vi "GpuMat IsContinuous.vi"(8 "error in (no error)":errorcluster, 11 "GpuMat in":refnum<class "GpuMat.lvclass">) -> (0 "error out":errorcluster, 2 "IsContinuous":bool, 3 "GpuMat out":refnum<class "GpuMat.lvclass">)   [LabVIEW 2020, in "OpenLvVision_OpenCv.lvlib" / "Cuda.lvlib" / "GpuMat.lvclass"]
doc: "Returns true if the GpuMat is stored contiguously (no padding/gaps between rows)."
uses:
  GpuMat.lvclass
  C:/Users/lukas/Documents/OpenLvVision_OpenCv/SourceCode/LabView/OpenLvVision_OpenCv/_LvHelpers/EdvrObject/EdvrObject.lvclass
  _LvHelpers/EdvrObject/EdvrObject.lvclass/EdvrObject.ctl
  OpenLvVision_OpenCv.lvlib
  <vilib>/Utility/error.llb/Error Cluster From Error Code.vi
  <vilib>/ErrorRing/Error Ring.xnode
  _LvHelpers/EdvrObject/EdvrObject.lvclass
  Dlls/OlvOpenCvWrapper.dll
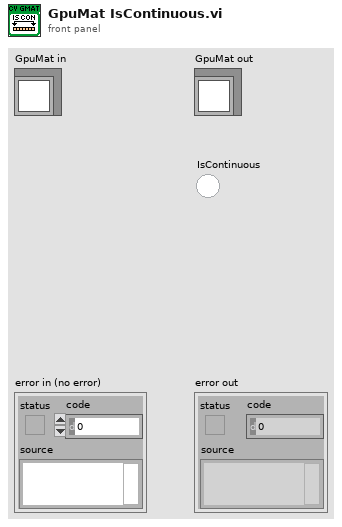
[diagram p1: front panel]
types:
  T1 = typedef "OpenLvVision_OpenCv.lvlib/EdvrObject.lvclass/Edvr.ctl" = refnum<data-value>
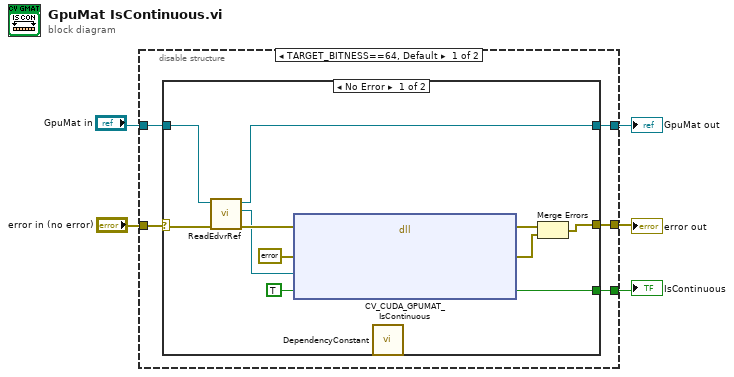
[diagram p0: block diagram]
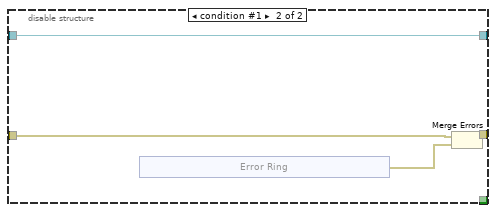
[diagram p3: hidden frame]
diagram:
  n1 = disable-structure shown="TARGET_BITNESS==64, Default" {
    disable-tunnel: "error in (no error)" -> [w10 w26]
    disable-tunnel: [w9 w27] -> w5
    disable-tunnel: "GpuMat in" -> [w8 w24]
    disable-tunnel: [w7 w24] -> w2
    disable-tunnel: [w6 _] -> w1
    frame condition #0 (active) {
      n2 = case shown="No Error" w10 {
        selector: w10 -> [w13 w23]
        tunnel: [w18 w23] -> w9
        tunnel: w8 -> [w16 w22]
        tunnel: [w14 w22] -> w7
        tunnel: [w12 _] -> w6
        frame No Error {
          n3 = call "ReadEdvrRef.vi"("error in (no error)"=w13, "EdvrObject in"=w16) -> ("error out"=w17:errorcluster, "Edvr"=w15:T1, "EdvrObject out"=w14:refnum<class "GpuMat.lvclass">)  [unwired: 7 in]
          n4 = dll-call lib="C:/Users/lukas/Documents/OpenLvVision_OpenCv/SourceCode/LabView/OpenLvVision_OpenCv/Dlls/OlvOpenCvWrapper.dll" fn="CV_CUDA_GPUMAT_IsContinuous"(error in=w17, "Error"=errorcluster {"status"=FALSE, "code"=0, "source"=""} ("error out"), "edvrRef"=w15, "result"=TRUE) -> (error out=w21:errorcluster, "Error"=w20:errorcluster, "result"=w12:bool)  [unwired: 4 in, 1 out]
          n5 = call "DependencyConstant.vi"() -> ()  [unwired: 12 in]
          n6 = Merge Errors(w21, w20) -> (w18:errorcluster)
        }
        frame Error {
        }
      }
    }
    frame condition #1 {
      n7 = xnode "Error Ring"() -> ("error out"=w25:errorcluster)
      n8 = Merge Errors(w26, w25) -> (w27:errorcluster)
    }
  }
  "error out" <- w5
  "GpuMat out" <- w2
  "IsContinuous" <- w1
